vi "02-sqrt_with_error_processing.vi"() -> ()   [LabVIEW 2018, in "LV2Julia_examples.lvlib"]
uses:
  LV2Julia_examples.lvlib
  LV2Julia_core/VIs/Server or client state.ctl
  LV2Julia_core/VIs/detailed error info.ctl
  LV2Julia_core/VIs/StackFrame.ctl
  LV2Julia_core/VIs/Commands.ctl
  71822543-7cbf-4033-aa74-7db116e85992.vi
  b897c894-e0b8-431a-8f01-351e2a203d12.vi
  58be0884-5f24-4db8-a231-ae1e3d7df6fe.vi
  <vilib>/Utility/High Resolution Relative Seconds.vi
  b897c894-e0b8-431a-8f01-351e2a203d12.vi/03462d35-fc46-426d-aa6d-e370c7a9654b.vi
  b897c894-e0b8-431a-8f01-351e2a203d12.vi/03462d35-fc46-426d-aa6d-e370c7a9654b.vi/c093fdcb-3a90-4f8f-8db8-3438935e1e44.vi
  b897c894-e0b8-431a-8f01-351e2a203d12.vi/03462d35-fc46-426d-aa6d-e370c7a9654b.vi/b0ce9ef7-e144-4a9e-9081-523436aa431f.vi
  b897c894-e0b8-431a-8f01-351e2a203d12.vi/03462d35-fc46-426d-aa6d-e370c7a9654b.vi/dc2cc107-4516-4618-a59f-0ec5ec480e68.vi
  LV2Julia_core/VIs/jl-scripts path.vi
  LV2Julia_core/VIs/check ID validity.vi
  LV2Julia_core/VIs/bindata_descr to JSON.vi
  LV2Julia_core/VIs/check cluster field names.vi
  LV2Julia_core/VIs/concat JSON.vi
  LV2Julia_core/VIs/build request.vi
  LV2Julia_core/VIs/Parse server response.vi
  LV2Julia_core/VIs/log jl exceptions.vi
  LV2Julia_core/LV2Julia_core.lvlib
panel:
  out "call duration (ms)":dbl format="%#.2f"
  in  "x":dbl=2.0
  in  "next":bool
  out "sqrt":dbl=nan
  out "detailed error info":T1
  out "current error":errorcluster
  out "final error":errorcluster
  out "short err code":u8
  in  "stop":bool
  out "ZMQ timeout":bool
  out "Julia script file path":path
  out "temporary script path":path
  out "Jl Server state":T3
  # "On a negative argument, an exception occurs in Julia. \n\nThe Julia server catches the exception and passes the information to the LV client:  Below you get detailed error information. The Jula server keeps running and is ready to process the next request. Note that error processing in Julia can be slow.\n\nThe last 1024 (you can change the number) exceptions in the current session are logged into the global \"jl stack traces global.vi\".  On exception, this VI opens the front panel of that global."
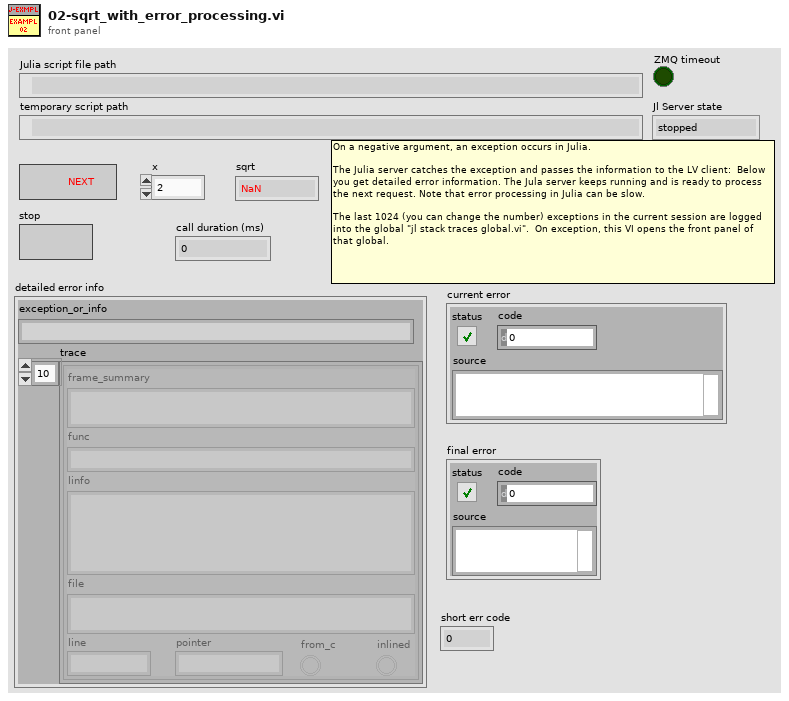
[diagram p1: front panel]
types:
  T1 = typedef "LV2Julia_core.lvlib/detailed error info.ctl" = cluster{"exception_or_info":string, "trace":T2[]}
  T2 = typedef "LV2Julia_core.lvlib/StackFrame.ctl" = cluster{"frame_summary":string, "func":string, "linfo":string, "file":string, "line":i32, "pointer":u64, "from_c":bool, "inlined":bool}
  T3 = typedef "LV2Julia_core.lvlib/Server or client state.ctl" = enum16{"stopped", "running", "unknown"}
  T4 = typedef "LV2Julia_core.lvlib/Commands.ctl" = enum16{"Start Jl-server & Init LV-client", "Send request & Get response ", "Stop Jl-server & Cleanup LV-client", "Cleanup LV-client", "Start Jl-server", "Stop Jl-server", "Init LV-Client", "Cleanup LV-Client", "(not allowed)", "Set LV Client state", "Set Jl Server state", "set ZMQ timeout", "read ZMQ timeout", "read-out state"}
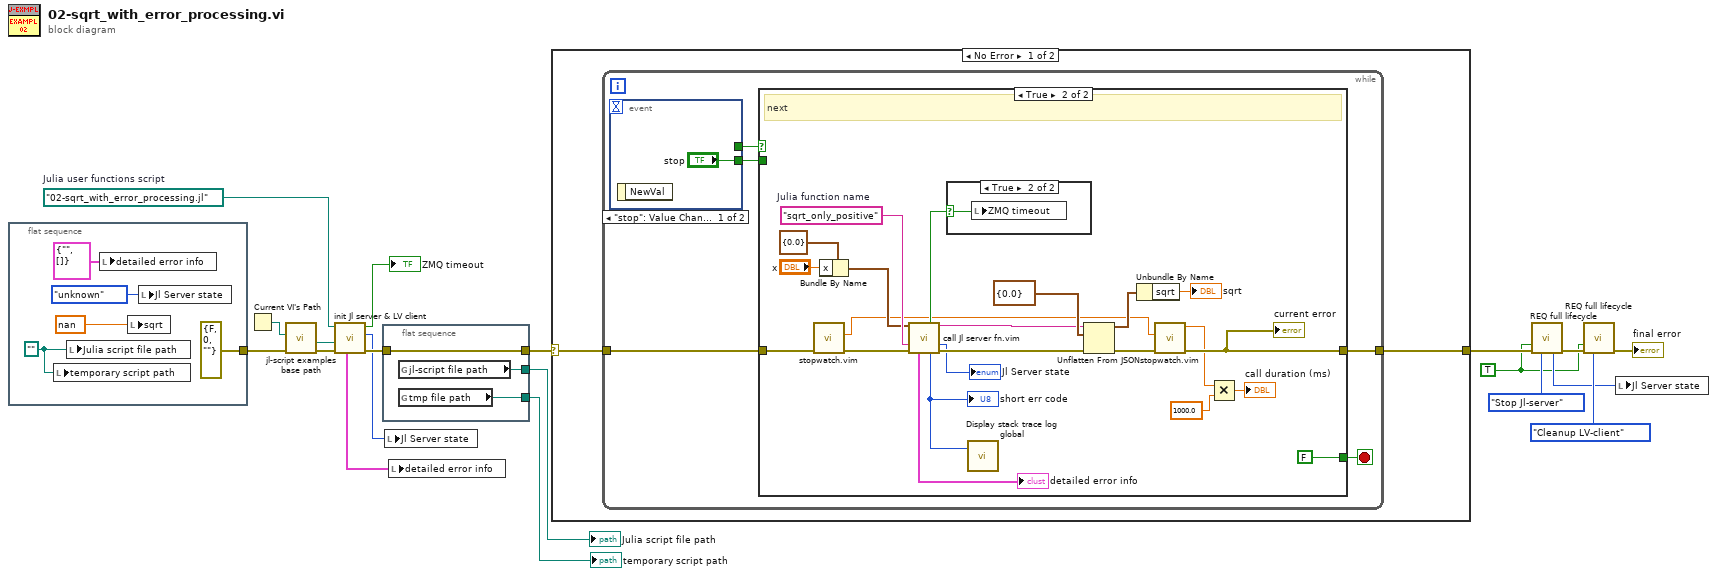
[diagram p0: block diagram]
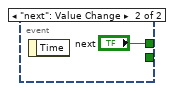
[diagram p2: hidden frame]
diagram:
  w9 = path "02-sqrt_with_error_processing.jl"  # Julia user functions script
  w10 = TRUE ("Force command")
  n1 = flat-sequence {
    tunnel: [errorcluster {"status"=FALSE, "code"=0, "source"=""} ("error in (no error)")] -> w4
    frame #0 {
      w20 = path ""
      n2 = local write "temporary script path"(w20) -> ()
      n3 = local write "Julia script file path"(w20) -> ()
      n4 = local write "detailed error info"(T1 {"exception_or_info"="", "trace"=[]} ("detailed error info")) -> ()
      n5 = local write "sqrt"(nan ("Server response")) -> ()
      n6 = local write "Jl Server state"(Server_or_client_state."unknown" ("Jl Server state out")) -> ()
    }
  }
  n7 = Current VI's Path() -> (path=w5:path)
  n8 = call "jl-script examples base path.vi"("error in (no error)"=w4, "calling example VI path"=w5) -> ("error out"=w3:errorcluster, "jl-script-examples base path"=w2:path)  [unwired: 8 in]
  n9 = call "init Jl server & LV client.vi"("error in (no error)"=w3, "Base path (not a path)"=w2, "Julia user functions script"=w9) -> ("error out"=w8:errorcluster, "Jl Server state out"=w6:T3, "timeout?"=→"ZMQ timeout":bool, "detailed error info"=w1:T1)  [unwired: 3 in, 2 out]
  n10 = flat-sequence {
    tunnel: [w27] -> w14
    tunnel: w8 -> [w27]
    tunnel: [w26] -> w12
    tunnel: [w25] -> w13
    frame #0 {
      n11 = global read "jl-scripts path.vi" "jl-script file path"() -> (w26:path)
      n12 = global read "jl-scripts path.vi" "tmp file path"() -> (w25:path)
    }
  }
  n13 = local write "Jl Server state"(w6) -> ()
  n14 = local write "detailed error info"(w1) -> ()
  n15 = case shown="No Error" w14 {
    selector: w14 -> [w28 w62]
    tunnel: [w29 w62] -> w19
    frame No Error {
      n16 = while {
        tunnel: w28 -> [w33]
        tunnel: [w34] -> w29
        stop <- w31 stop-if-true
        n17 = event shown="[0] \"stop\": Value Change" {
          selector: _ -> [_ _]
          dyn-events: _ -> [_ _]
          timeout: _ -> [_ _]
          tunnel: [_ "next"] -> w32
          tunnel: ["stop" _] -> w30
          event "stop": Value Change {
            n18 = event-data() -> ()  [unwired: 1 in, 1 out]
          }
          event "next": Value Change {
            n19 = event-data() -> ()  [unwired: 1 in, 1 out]
          }
        }
        n20 = case shown="True" w32 {
          tunnel: [w38 w41] -> w34
          tunnel: w33 -> [w38 w44]
          tunnel: [w37 FALSE ("stop this VI only")] -> w31
          tunnel: w30 -> [w37 _]
          frame False {
            # "stop"
          }
          frame True {
            w53 = "sqrt_only_positive"  # Julia function name
            # "next"
            n21 = call "stopwatch.vim"("anything in"=w44) -> ("copy of anything out"=w43:errorcluster, "current timepoint"=w40:dbl)  [unwired: 8 in, 1 out]
            n22 = Bundle By Name(cluster=cluster{"x":dbl} {"x"=0.0}, "x"="x") -> (w52:cluster{"x":dbl})
            n23 = call "call Jl server fn.vim"("Arguments 1"=w52, "fun2call"=w53, "error in (no error)"=w43) -> ("timeout?"=w49:bool, "JSON received"=w48:string, "Jl Server state out"=→"Jl Server state":T3, "detailed error info"=→"detailed error info":T1, "return code"=w47:u8, "error out"=w54:errorcluster)  [unwired: 6 in, 1 out]
            "short err code" <- w47
            n24 = case shown="True" w49 {
              selector: w49 -> [_ w61]
              frame False {
              }
              frame True {
                n25 = local write "ZMQ timeout"(w61) -> ()
              }
            }
            n26 = call "Display stack trace log global.vi"("server return code"=w47) -> ()  [unwired: 3 in]
            n27 = Unflatten From JSON(JSON string=w48, type and defaults=cluster{"sqrt":dbl} {"sqrt"=0.0} ("parsed response"), error in (no error)=w54) -> (value=w59:cluster{"sqrt":dbl}, error out=w42:errorcluster)  [unwired: 4 in]
            n28 = Unbundle By Name(w59) -> ("sqrt"=→"sqrt":dbl)
            n29 = call "stopwatch.vim"("anything in"=w42, "prev timepoint (0)"=w40) -> ("copy of anything out"=w41:errorcluster, "delta t (s)"=w39:dbl)  [unwired: 7 in, 1 out]
            "current error" <- w41
            n30 = Multiply(x=w39, y=1000.0) -> (x*y=→"call duration (ms)":dbl)
          }
        }
      }
    }
    frame Error {
    }
  }
  n31 = call "REQ full lifecycle.vi"("Force command"=w10, "error in"=w19, "command"=Commands."Stop Jl-server") -> ("Jl Server state out"=w11:T3, "error out"=w17:errorcluster)  [unwired: 6 in, 5 out]
  n32 = call "REQ full lifecycle.vi"("Force command"=w10, "error in"=w17, "command"=Commands."Cleanup LV-client") -> ("error out"=→"final error":errorcluster)  [unwired: 6 in, 6 out]
  n33 = local write "Jl Server state"(w11) -> ()
  "temporary script path" <- w13
  "Julia script file path" <- w12
